vi "VIH Utility - MENU - Create Menu.vi"   [LabVIEW 2014]
doc: "::: VI Helpeks :::\nCopyright (c) 2000-2026 Konstantin Shifershteyn. All rights reserved."
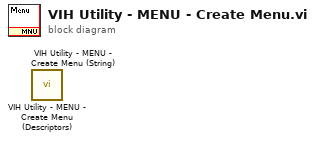
[diagram p0: block diagram]
diagram:
  n1 = call "VIH Utility - MENU - Create Menu (Descriptors).vi"() -> ()  [unwired: 10 in, 2 out]
  n2 = call "VIH Utility - MENU - Create Menu (String).vi"() -> ()  [unwired: 10 in, 2 out]
